vi "sandbox xpub sub.vi"() -> ()   [LabVIEW 2019, in "XPUB.lvclass"]
uses:
  XPUB.lvclass
  <vilib>/addons/zeromq/socket_type.ctl
  <vilib>/addons/zeromq/socket_options.ctl
  <vilib>/numeric/Random Number (Range) DBL.vi
  <vilib>/numeric/Random Number (Range) U64.vi
  9c8e6f28-ceda-4605-9ac7-498f97c638f3.vi
  <vilib>/numeric/sub_Random U32.vi
  <vilib>/JDP Science/JSONtext/Variant to JSON Text.vi
  <vilib>/JDP Science/JSONtext/Set Item.vi
  <vilib>/JDP Science/JSONtext/LVClass Serializer/JSONtext LVClass Serializer.lvclass
  <vilib>/addons/zeromq/zeromq.lvlib
  <vilib>/addons/zeromq/zmq_socket.lvclass
  <vilib>/addons/zeromq/zmq_context.lvclass
panel:
  out "xpub recv":string[](array[string])
  in  "pub topics":T1(ring)
  in  "sub topic":string
  in  "stop":bool
  in  "close":bool
  out "received":string[](array[string])
  out "sent":string[](array[string])
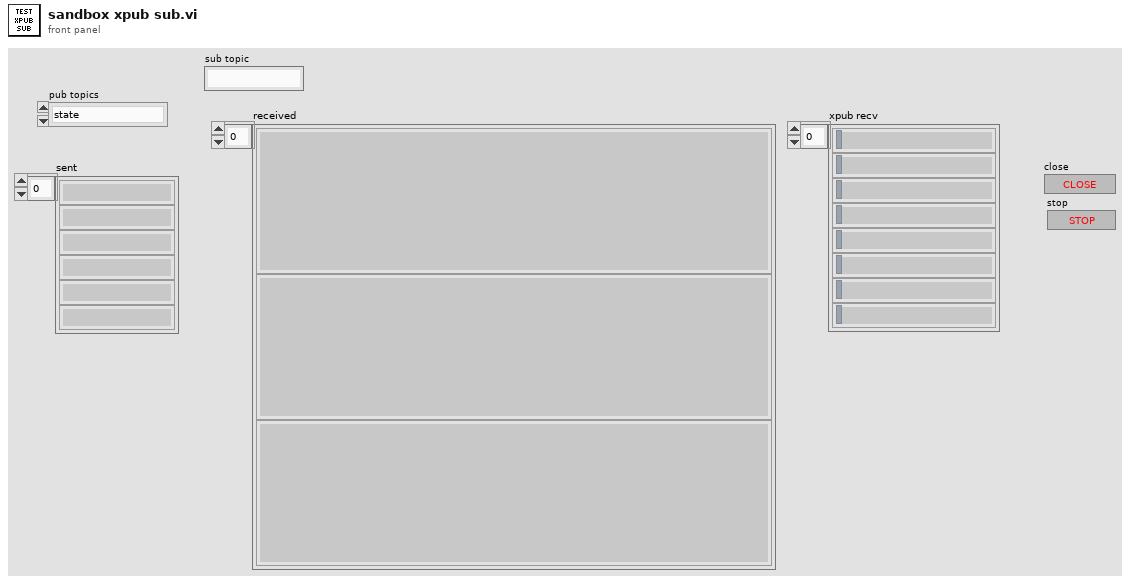
[diagram p1: front panel]
types:
  T1 = enum16{"state", "results", "waveforms.ai", "waveforms.ao", "sweep.ai", "sweep.ao", "sweep.x", "sweep.y"}
  T2 = typedef "zeromq.lvlib/socket_type.ctl" = enum8{"ZMQ_PAIR", "ZMQ_PUB", "ZMQ_SUB", "ZMQ_REQ", "ZMQ_REP", "ZMQ_DEALER", "ZMQ_ROUTER", "ZMQ_PULL", "ZMQ_PUSH", "ZMQ_XPUB", "ZMQ_XSUB", "ZMQ_STREAM", "ZMQ_SERVER", "ZMQ_CLIENT", "ZMQ_RADIO", "ZMQ_DISH", "ZMQ_GATHER", "ZMQ_SCATTER", "ZMQ_DGRAM"}
  T3 = cluster{"number":u64, "number":dbl, "string":string}
  T4 = typedef "zeromq.lvlib/socket_options.ctl" = enum8{"NONE", "ZMQ_HWM", "<2>", "ZMQ_SWAP", "ZMQ_AFFINITY", "ZMQ_ROUTING_ID", "ZMQ_SUBSCRIBE", "ZMQ_UNSUBSCRIBE", "ZMQ_RATE", "ZMQ_RECOVERY_IVL", "ZMQ_MCAST_LOOP", "ZMQ_SNDBUF", "ZMQ_RCVBUF", "ZMQ_RCVMORE", "ZMQ_FD", "ZMQ_EVENTS", "ZMQ_TYPE", "ZMQ_LINGER", "ZMQ_RECONNECT_IVL", "ZMQ_BACKLOG", "ZMQ_RECOVERY_IVL_MSEC", "ZMQ_RECONNECT_IVL_MAX", "ZMQ_MAXMSGSIZE", "ZMQ_SNDHWM", "ZMQ_RCVHWM", "ZMQ_MULTICAST_HOPS", "<26>", "ZMQ_RCVTIMEO", "ZMQ_SNDTIMEO", "<29>", "<30>", "ZMQ_IPV4ONLY", "ZMQ_LAST_ENDPOINT", "ZMQ_ROUTER_MANDATORY", "ZMQ_TCP_KEEPALIVE", "ZMQ_TCP_KEEPALIVE_CNT", "ZMQ_TCP_KEEPALIVE_IDLE", "ZMQ_TCP_KEEPALIVE_INTVL", "ZMQ_TCP_ACCEPT_FILTER", "ZMQ_IMMEDIATE", "ZMQ_XPUB_VERBOSE", "ZMQ_ROUTER_RAW", "ZMQ_IPV6", "ZMQ_MECHANISM", "ZMQ_PLAIN_SERVER", "ZMQ_PLAIN_USERNAME", "ZMQ_PLAIN_PASSWORD", "ZMQ_CURVE_SERVER", "ZMQ_CURVE_PUBLICKEY", "ZMQ_CURVE_SECRETKEY", "ZMQ_CURVE_SERVERKEY", "ZMQ_PROBE_ROUTER", "ZMQ_REQ_CORRELATE", "ZMQ_REQ_RELAXED", "ZMQ_CONFLATE", "ZMQ_ZAP_DOMAIN", "ZMQ_ROUTER_HANDOVER", "ZMQ_TOS", "ZMQ_IPC_FILTER_PID", "ZMQ_IPC_FILTER_UID", "ZMQ_IPC_FILTER_GID", "ZMQ_CONNECT_ROUTING_ID", "ZMQ_GSSAPI_SERVER", "ZMQ_GSSAPI_PRINCIPAL", "ZMQ_GSSAPI_SERVICE_PRINCIPAL", "ZMQ_GSSAPI_PLAINTEXT", "ZMQ_HANDSHAKE_IVL", "<67>", "ZMQ_SOCKS_PROXY", "ZMQ_XPUB_NODROP", "ZMQ_BLOCKY", "ZMQ_XPUB_MANUAL", "ZMQ_XPUB_WELCOME_MSG", "ZMQ_STREAM_NOTIFY", "ZMQ_INVERT_MATCHING", "ZMQ_HEARTBEAT_IVL", "ZMQ_HEARTBEAT_TTL", "ZMQ_HEARTBEAT_TIMEOUT", "ZMQ_XPUB_VERBOSER", "ZMQ_CONNECT_TIMEOUT", "ZMQ_TCP_MAXRT", "ZMQ_THREAD_SAFE", "<82>", "<83>", "ZMQ_MULTICAST_MAXTPDU", "ZMQ_VMCI_BUFFER_SIZE", "ZMQ_VMCI_BUFFER_MIN_SIZE", "ZMQ_VMCI_BUFFER_MAX_SIZE", "ZMQ_VMCI_CONNECT_TIMEOUT", "ZMQ_USE_FD", "ZMQ_GSSAPI_PRINCIPAL_NAMETYPE", "ZMQ_GSSAPI_SERVICE_PRINCIPAL_NAMETYPE", "ZMQ_BINDTODEVICE", "ZMQ_ZAP_ENFORCE_DOMAIN", "ZMQ_LOOPBACK_FASTPATH", "ZMQ_METADATA", "ZMQ_MULTICAST_LOOP", "ZMQ_ROUTER_NOTIFY"}
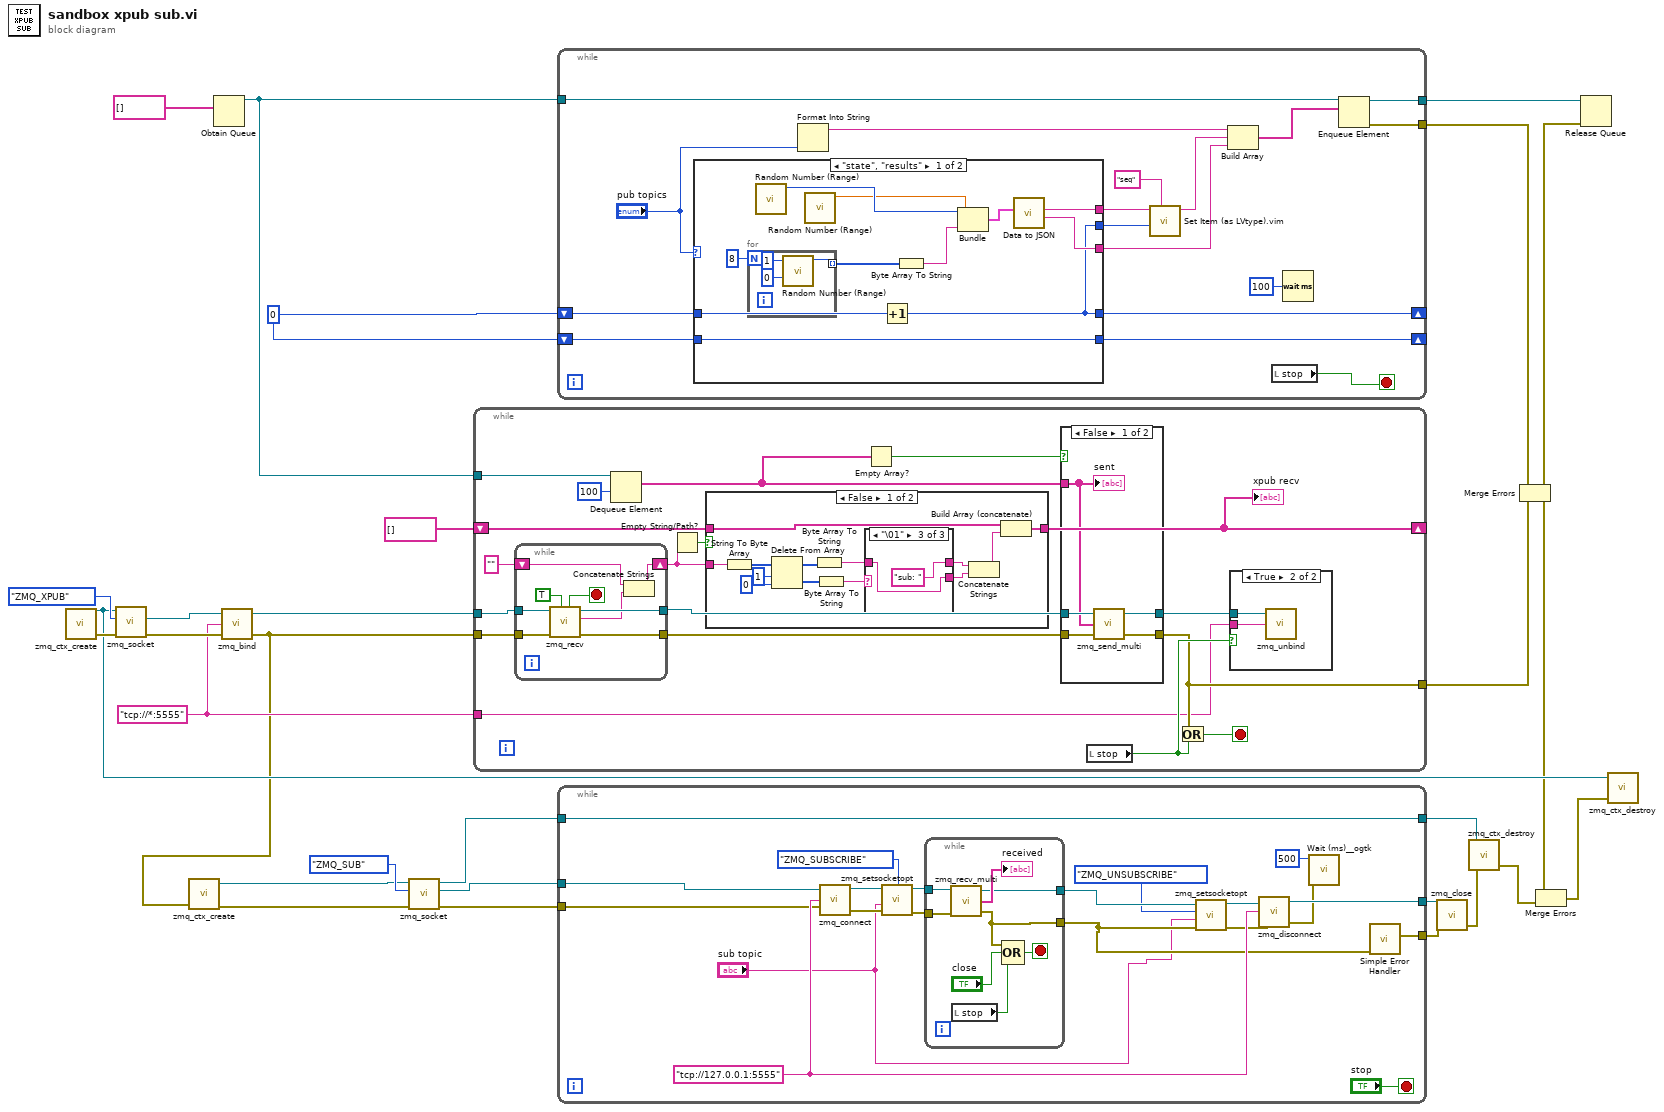
[diagram p0: block diagram]
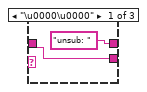
[diagram p2: hidden frame]
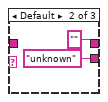
[diagram p3: hidden frame]
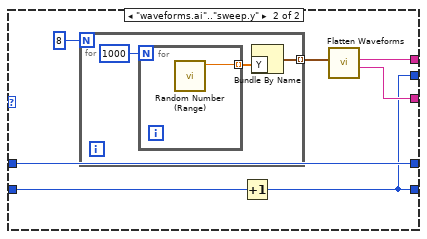
[diagram p7: hidden frame]
diagram:
  w21 = u64 0 ("lower bound (0)")
  w17 = "tcp://*:5555" ("endpoint")
  n1 = call <vilib>:"zmq_ctx_create.vi"() -> ("error out"=w27:errorcluster, "context out"=w20:refnum<class "zmq_context.lvclass">)  [unwired: 4 in]
  n2 = call <vilib>:"zmq_socket.vi"("error in"=w27, "socket type"=socket_type."ZMQ_XPUB", "context in"=w20) -> ("error out"=w26:errorcluster, "socket out"=w14:refnum<class "zmq_socket.lvclass">)  [unwired: 2 in, 1 out]
  n3 = Obtain Queue(element data type=string[] [] ("appended array")) -> (queue out=w23:refnum<queue>)  [unwired: 4 in, 2 out]
  n4 = call <vilib>:"zmq_bind.vi"("error in"=w26, "endpoint"=w17, "socket in"=w14) -> ("error out"=w13:errorcluster, "socket out"=w25:refnum<class "zmq_socket.lvclass">)  [unwired: 1 in]
  n5 = call <vilib>:"zmq_ctx_create.vi"("error in"=w13) -> ("error out"=w3:errorcluster, "context out"=w6:refnum<class "zmq_context.lvclass">)  [unwired: 3 in]
  n6 = call <vilib>:"zmq_socket.vi"("error in"=w3, "socket type"=socket_type."ZMQ_SUB", "context in"=w6) -> ("error out"=w2:errorcluster, "socket out"=w4:refnum<class "zmq_socket.lvclass">, "context out"=w5:refnum<class "zmq_context.lvclass">)  [unwired: 2 in]
  n7 = while {
    tunnel: w25 -> [w45]
    tunnel: w13 -> [w44]
    tunnel: w23 -> [w42]
    tunnel: [w37] -> w16
    tunnel: w17 -> [w36]
    shift-right: [w30] -> _
    shift-left: string[] [] -> [w33]
    stop <- w46 stop-if-true
    n8 = while {
      tunnel: w45 -> [w83]
      tunnel: [w81] -> w29
      tunnel: w44 -> [w80]
      tunnel: [w79] -> w43
      shift-right: [w76] -> w31
      shift-left: "" -> [w78]
      stop <- w82 stop-if-true
      n9 = call <vilib>:"zmq_recv.vi"("no block? (F)"=TRUE, "error in"=w80, "socket in"=w83) -> ("error out"=w79:errorcluster, "data"=w77:string, "socket out"=w81:refnum<class "zmq_socket.lvclass">, "timeout?"=w82:bool)  [unwired: 2 in, 1 out]
      n10 = Concatenate Strings(w78, w77) -> (w76:string)
    }
    n11 = Dequeue Element(queue=w42, timeout in ms (-1)=100) -> (element=w35:string[])  [unwired: 1 in, 3 out]
    n12 = Empty String/Path?(string/path=w31) -> (empty?=w32:bool)
    n13 = case shown="False" w32 {
      tunnel: w33 -> [w59 w66]
      tunnel: w31 -> [w58 _]
      tunnel: [w57 w66] -> w30
      frame False {
        n14 = String To Byte Array(string=w58) -> (unsigned byte array=w56:u8[])
        n15 = Delete From Array(array=w56, length=1, index=0) -> (deleted portion=w52:u8[], array with subset deleted=w53:u8[])
        n16 = Byte Array To String(unsigned byte array=w53) -> (string=w47:string)
        n17 = Byte Array To String(unsigned byte array=w52) -> (string=w51:string)
        n18 = case shown="\"\\01\"" w51 {
          tunnel: [w60 "unknown" w65] -> w49
          tunnel: ["unsub: " "" ("string") "sub: "] -> w48
          tunnel: w47 -> [w60 _ w65]
          frame "\u0000\u0000" {
          }
          frame Default {
          }
          frame "\u0001" {
          }
        }
        n19 = Concatenate Strings(w48, w49) -> (w50:string)
        n20 = Build Array (concatenate)(w59, w50) -> (w57:string[])
      }
      frame True {
      }
    }
    "xpub recv" <- w30
    n21 = Empty Array?(array=w35) -> (empty?=w40:bool)
    n22 = case shown="False" w40 {
      tunnel: [w73 w75] -> w37
      tunnel: w29 -> [w72 w74]
      tunnel: w43 -> [w71 w75]
      tunnel: w35 -> [w70 _]
      tunnel: [w69 w74] -> w39
      frame False {
        n23 = call <vilib>:"zmq_send_multi.vi"("error in"=w71, "parts"=w70, "socket in"=w72) -> ("error out"=w73:errorcluster, "socket out"=w69:refnum<class "zmq_socket.lvclass">)  [unwired: 1 in]
        "sent" <- w70
      }
      frame True {
      }
    }
    n24 = local read "stop"() -> (w38:bool)
    n25 = Or(x=w37, y=w38) -> (x .or. y?=w46:bool)
    n26 = case shown="True" w38 {
      tunnel: w39 -> [_ w68]
      tunnel: w36 -> [_ w67]
      frame False {
      }
      frame True {
        n27 = call <vilib>:"zmq_unbind.vi"("endpoint"=w67, "socket in"=w68) -> ()  [unwired: 2 in, 2 out]
      }
    }
  }
  n28 = while {
    tunnel: w23 -> [w101]
    tunnel: [w93] -> w22
    shift-right: [w89] -> _
    shift-left: w21 -> [w92]
    shift-right: [w88] -> _
    shift-left: w21 -> [w91]
    tunnel: [w86] -> w19
    stop <- w95 stop-if-true
    n29 = case shown="\"state\", \"results\"" "pub topics" {
      tunnel: [w111 w122] -> w99
      tunnel: [w112 w121] -> w98
      tunnel: w92 -> [w104 w118]
      tunnel: w91 -> [w102 w117]
      tunnel: [w103 w116] -> w90
      tunnel: [w103 w118] -> w89
      tunnel: [w102 w116] -> w88
      frame "state", "results" {
        n30 = for {
          N: 8 -> [_]
          tunnel: [w115] -> w105 mode=indexing
          n31 = call-poly <vilib>:"Random Number (Range).vi"("lower bound (0)"=u64 0, "upper bound (100)"=u64 1) -> ("number"=w115:u64)  [unwired: 9 in]
        }
        n32 = call-poly <vilib>:"Random Number (Range).vi"() -> ("number"=w110:u64)  [unwired: 11 in]
        n33 = call-poly <vilib>:"Random Number (Range).vi"() -> ("number"=w108:dbl)  [unwired: 11 in]
        n34 = Increment(x=w104) -> (x+1=w103:u64)
        n35 = Byte Array To String(unsigned byte array=w105) -> (string=w107:string)
        n36 = Bundle("number"=w110, "number"=w108, "string"=w107) -> (w109:T3)  [unwired: 1 in]
        n37 = call "Data to JSON.vi"("Data in"=w109) -> ("<JSON> data"=w111:string, "<JSON> header"=w112:string)  [unwired: 8 in, 1 out]
      }
      frame "waveforms.ai".."sweep.y" {
        n38 = for {
          N: 8 -> [_]
          tunnel: [w124] -> w119 mode=indexing
          n39 = for {
            N: 1000 -> [_]
            tunnel: [w126] -> w125 mode=indexing
            n40 = call-poly <vilib>:"Random Number (Range).vi"() -> ("number"=w126:dbl)  [unwired: 11 in]
          }
          n41 = Bundle By Name("Y"=w125) -> (w124:waveform(dbl))  [unwired: 1 in]
        }
        n42 = Increment(x=w117) -> (x+1=w116:u64)
        n43 = call "Flatten Waveforms.vi"("Waveforms in"=w119) -> ("flattened data"=w122:string, "<JSON> header"=w121:string)  [unwired: 8 in, 1 out]
      }
    }
    n44 = Format Into String("pub topics") -> (resulting string=w100:string)  [unwired: 3 in, 1 out]
    n45 = call "Set Item (as LVtype).vim"("$Path or Item Name"="seq", "Anything"=w90, "JSON"=w98) -> ("<JSON>"=w97:string)  [unwired: 5 in, 2 out]
    n46 = Build Array(w100, w97, w99) -> (w94:string[])
    n47 = local read "stop"() -> (w95:bool)
    n48 = Wait (ms)(milliseconds to wait=u32 100) -> ()  [unwired: 1 out]
    n49 = Enqueue Element(queue=w101, element=w94) -> (queue out=w93:refnum<queue>, error out=w86:errorcluster)  [unwired: 2 in, 1 out]
  }
  n50 = while {
    tunnel: [w139] -> w11
    tunnel: [w138] -> w10
    tunnel: w4 -> [w130]
    tunnel: [w132] -> w12
    tunnel: w5 -> [w132]
    tunnel: w2 -> [w131]
    stop <- "stop" stop-if-true
    w140 = "tcp://127.0.0.1:5555" ("endpoint")
    n51 = call <vilib>:"zmq_connect.vi"("error in"=w131, "endpoint"=w140, "socket in"=w130) -> ("error out"=w145:errorcluster, "socket out"=w146:refnum<class "zmq_socket.lvclass">)  [unwired: 1 in]
    n52 = call <vilib>:"zmq_setsocketopt.vi"("error in"=w145, "value"="sub topic", "option"=socket_options."ZMQ_SUBSCRIBE", "socket in"=w146) -> ("error out"=w144:errorcluster, "socket out"=w143:refnum<class "zmq_socket.lvclass">)  [unwired: 2 in]
    n53 = while {
      tunnel: w143 -> [w154]
      tunnel: w144 -> [w152]
      tunnel: [w149] -> w134
      tunnel: [w148] -> w137
      stop <- w150 stop-if-true
      n54 = call <vilib>:"zmq_recv_multi.vi"("error in"=w152, "socket in"=w154) -> ("error out"=w149:errorcluster, "parts"=→"received":string[], "socket out"=w148:refnum<class "zmq_socket.lvclass">)  [unwired: 1 in]
      n55 = local read "stop"() -> (w147:bool)
      n56 = Compound Arithmetic op=OR(w149, "close", w147) -> (w150:bool)
    }
    n57 = call <vilib>:"zmq_setsocketopt.vi"("error in"=w134, "value"="sub topic", "option"=socket_options."ZMQ_UNSUBSCRIBE", "socket in"=w137) -> ("error out"=w133:errorcluster, "socket out"=w135:refnum<class "zmq_socket.lvclass">)  [unwired: 2 in]
    n58 = call <vilib>:"zmq_disconnect.vi"("error in"=w133, "endpoint"=w140, "socket in"=w135) -> ("error out"=w128:errorcluster, "socket out"=w139:refnum<class "zmq_socket.lvclass">)  [unwired: 1 in]
    n59 = call <userlib>:"Wait (ms)__ogtk.vi"("error in (no error)"=w128, "milliseconds to wait"=u32 500) -> ()  [unwired: 8 in, 2 out]
    n60 = call <vilib>:"Simple Error Handler.vi"("error in (no error)"=w134) -> ("error out"=w138:errorcluster)  [unwired: 4 in, 4 out]
  }
  n61 = call <vilib>:"zmq_close.vi"("error in"=w10, "socket"=w11) -> ("error out"=w9:errorcluster)  [unwired: 3 in]
  n62 = call <vilib>:"zmq_ctx_destroy.vi"("error in"=w9, "context in"=w12) -> ("error out"=w8:errorcluster)  [unwired: 3 in]
  n63 = Merge Errors(w19, w16) -> (w15:errorcluster)
  n64 = Merge Errors(w15, w8) -> (w18:errorcluster)
  n65 = Release Queue(queue=w22, error in (no error)=w15) -> ()  [unwired: 1 in, 3 out]
  n66 = call <vilib>:"zmq_ctx_destroy.vi"("error in"=w18, "context in"=w20) -> ()  [unwired: 3 in, 1 out]
